vi "UMLEditor loadIniFileInfo.vi"(1 "menu":refnum<k9>, 2 "iniFile":path, 5 "error in (no error)":errorcluster) -> (11 "StabilityProblems":bool, 13 "SyncTime":u32, 15 "Ini-FileFound":bool, 16 "ToolHelp":bool, 17 "LastDiagramType":T1, 18 "FileToOpen":path, 19 "error out":errorcluster)   [LabVIEW 2020]
doc: "Gets current diagram values"
uses:
  <resource>/Framework/Providers/Open_GDS/UML/UMLEditor/UMLEditor_DiagramType.ctl
  <resource>/Framework/Providers/Open_GDS/UML/UMLEditor/UMLEditor_SyncOptions.ctl
  <resource>/Framework/Providers/Open_GDS/UML/UMLEditor/UMLEditor_IniFileData.ctl
  <resource>/Framework/Providers/Open_GDS/UML/UMLEditor/UMLEditor_StoredPathes.ctl
  <resource>/Framework/Providers/Open_GDS/ClassProviders/Common/File/File_StoredPathesActions.ctl
  <resource>/Framework/Providers/Open_GDS/UML/UMLEditor/UMLEditor_StoredColors.ctl
  <resource>/Framework/Providers/Open_GDS/UML/UmlEditor_class/IniParamsType.ctl
  <resource>/Framework/Providers/Open_GDS/ClassProviders/Common/CommonVIs/CommonVIs_ColorMemoryAction.ctl
  <resource>/Framework/Providers/Open_GDS/UML/UMLEditor/UMLEditor MenuActionType.ctl
  <resource>/Framework/Providers/Open_GDS/UML/UmlEditor_class/UmlEditor.lvclass
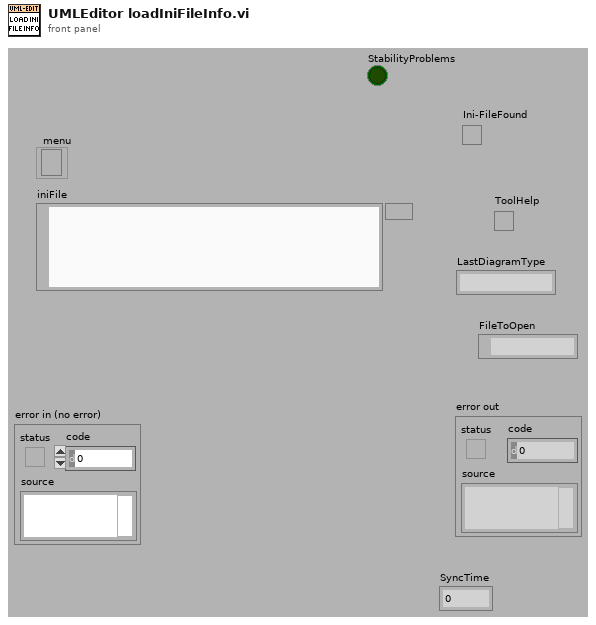
[diagram p1: front panel]
types:
  T1 = typedef "UMLEditor_DiagramType.ctl" = string
  T2 = typedef "UMLEditor_SyncOptions.ctl" = cluster{"IgnoreInstrLib":bool, "IgnoreUserLib":bool, "IgnoreViLib":bool}
  T3 = cluster{"RecentFiles":string[], "LastDiagramType":T1, "ShowToolHelp":bool, "Paths":cluster{"LastSerachPath":path, "QueuedArrayStateVI":path, "ClassBasePath":path, "VITemplatePath":path, "ApplicationTemplatePath":path, "RevPlugIns":path}, "Colors":cluster{"ClassBackgroudColor":u32, "ClassBackgroudColorWithClassPath":u32, "ClassBackgroudColorForApplicationVIStereotype":u32, "ClassBackgroudColorForTypeStereotype":u32, "StateBackgroudColor":u32}, "ProjectBaseClassOption":bool, "CreateTypesWhenSynchronizing":bool, "AttributeToIgnoreInSync":string[], "ToolTip":cluster{"ToolTipOpen":bool, "LastToolTip":i32}, "ClassesToIgnoreInSync":string[], "UndoSize":i32, "OpenLastSavedFile":bool, "SyncOption":T2, "SyncTime":u32, "Params":cluster{"Name":string, "Value":string}[]}
  T4 = typedef "UMLEditor_IniFileData.ctl" = cluster{"RecentFiles":string[], "LastDiagramType":T1, "ShowToolHelp":bool, "Paths":cluster{"LastSerachPath":path, "QueuedArrayStateVI":path, "ClassBasePath":path, "VITemplatePath":path, "ApplicationTemplatePath":path, "RevPlugIns":path}, "Colors":cluster{"ClassBackgroudColor":u32, "ClassBackgroudColorWithClassPath":u32, "ClassBackgroudColorForApplicationVIStereotype":u32, "ClassBackgroudColorForTypeStereotype":u32, "StateBackgroudColor":u32, "ClassBackgroudColorForApplicationInterfaceStereotype":u32}, "ProjectBaseClassOption":bool, "CreateTypesWhenSynchronizing":bool, "AttributeToIgnoreInSync":string[], "ToolTip":cluster{"ToolTipOpen":bool, "LastToolTip":i32}, "ClassesToIgnoreInSync":string[], "UndoSize":i32, "OpenLastSavedFile":bool, "SyncOption":T2, "SyncTime":u32, "Params":cluster{"Name":string, "Value":string}[]}
  T5 = cluster{"RecentFiles":string[], "LastDiagramType":T1, "ShowToolHelp":bool, "Paths":cluster{"LastSerachPath":path, "QueuedArrayStateVI":path, "ClassBasePath":path, "VITemplatePath":path, "ApplicationTemplatePath":path, "RevPlugIns":path}, "Colors":cluster{"ClassBackgroudColor":u32, "ClassBackgroudColorWithClassPath":u32, "ClassBackgroudColorForApplicationVIStereotype":u32, "ClassBackgroudColorForTypeStereotype":u32, "StateBackgroudColor":u32}, "ProjectBaseClassOption":bool, "CreateTypesWhenSynchronizing":bool, "AttributeToIgnoreInSync":string[], "ToolTip":cluster{"ToolTipOpen":bool, "LastToolTip":i32}, "ClassesToIgnoreInSync":string[], "UndoSize":i32, "OpenLastSavedFile":bool, "SyncOption":T2}
  T6 = cluster{"RecentFiles":string[], "LastDiagramType":T1, "ShowToolHelp":bool, "Paths":cluster{"LastSerachPath":path, "QueuedArrayStateVI":path, "ClassBasePath":path, "VITemplatePath":path, "ApplicationTemplatePath":path, "RevPlugIns":path}, "Colors":cluster{"ClassBackgroudColor":u32, "ClassBackgroudColorWithClassPath":u32, "ClassBackgroudColorForApplicationVIStereotype":u32, "ClassBackgroudColorForTypeStereotype":u32, "StateBackgroudColor":u32}, "ProjectBaseClassOption":bool, "CreateTypesWhenSynchronizing":bool, "AttributeToIgnoreInSync":string[], "ToolTip":cluster{"ToolTipOpen":bool, "LastToolTip":i32}, "ClassesToIgnoreInSync":string[], "UndoSize":i32}
  T7 = cluster{"RecentFiles":string[], "LastDiagramType":T1, "ShowToolHelp":bool, "Paths":cluster{"LastSerachPath":path, "QueuedArrayStateVI":path, "ClassBasePath":path, "VITemplatePath":path, "ApplicationTemplatePath":path, "RevPlugIns":path}, "Colors":cluster{"ClassBackgroudColor":u32, "ClassBackgroudColorWithClassPath":u32, "ClassBackgroudColorForApplicationVIStereotype":u32, "ClassBackgroudColorForTypeStereotype":u32, "StateBackgroudColor":u32}, "ProjectBaseClassOption":bool, "CreateTypesWhenSynchronizing":bool, "AttributeToIgnoreInSync":string[], "ToolTip":cluster{"ToolTipOpen":bool, "LastToolTip":i32}, "ClassesToIgnoreInSync":string[], "UndoSize":i32, "OpenLastSavedFile":bool, "SyncOption":T2, "SyncTime":u32}
  T8 = typedef "UmlEditor.lvclass/IniParamsType.ctl" = enum16{"I have problem with UML stability on my computer"}
  T9 = typedef "UMLEditor_StoredColors.ctl" = enum16{"ClassBackgroudColor", "ClassBackgroudColorWithClassPath", "ClassBackgroudColorForApplicationVIStereotype", "ClassBackgroudColorForTypeStereotype", "StateBackgroudColor", "ClassBackgroudColorForInterfaceStereotype"}
  T10 = typedef "UMLEditor_StoredPathes.ctl" = enum16{"LastSearchPath", "QueuedArrayStateVI", "ClassBasePath", "ViTemplatePath", "ApplicationTemplatePath", "IniFilePath", "WizDir", "RevPlugInPath"}
  T11 = typedef "UMLEditor MenuActionType.ctl" = enum16{"EnableSave", "EnablePaste", "DisablePaste", "DiableSave", "AddRecentFile", "disablePropDel", "enablePropDel", "enablePropDisDel", "diasbleClassRel", "enableClassRel", "Class", "State", "Other", "EnableXMI", "DisableXMI", "EnableCopy", "DisableCopy"}
  T12 = typedef "CommonVIs_ColorMemoryAction.ctl" = enum16{"Get Color", "Set Color", "Delete Color", "Clear All Colors"}
  T13 = typedef "File_StoredPathesActions.ctl" = enum16{"Get Path", "Set Path", "Delete Path", "Clear All Paths"}
  T14 = cluster{"LastSerachPath":path, "QueuedArrayStateVI":path, "ClassBasePath":path, "VITemplatePath":path, "ApplicationTemplatePath":path, "RevPlugIns":path}
  T15 = cluster{"ClassBackgroudColor":u32, "ClassBackgroudColorWithClassPath":u32, "ClassBackgroudColorForApplicationVIStereotype":u32, "ClassBackgroudColorForTypeStereotype":u32, "StateBackgroudColor":u32, "ClassBackgroudColorForApplicationInterfaceStereotype":u32}
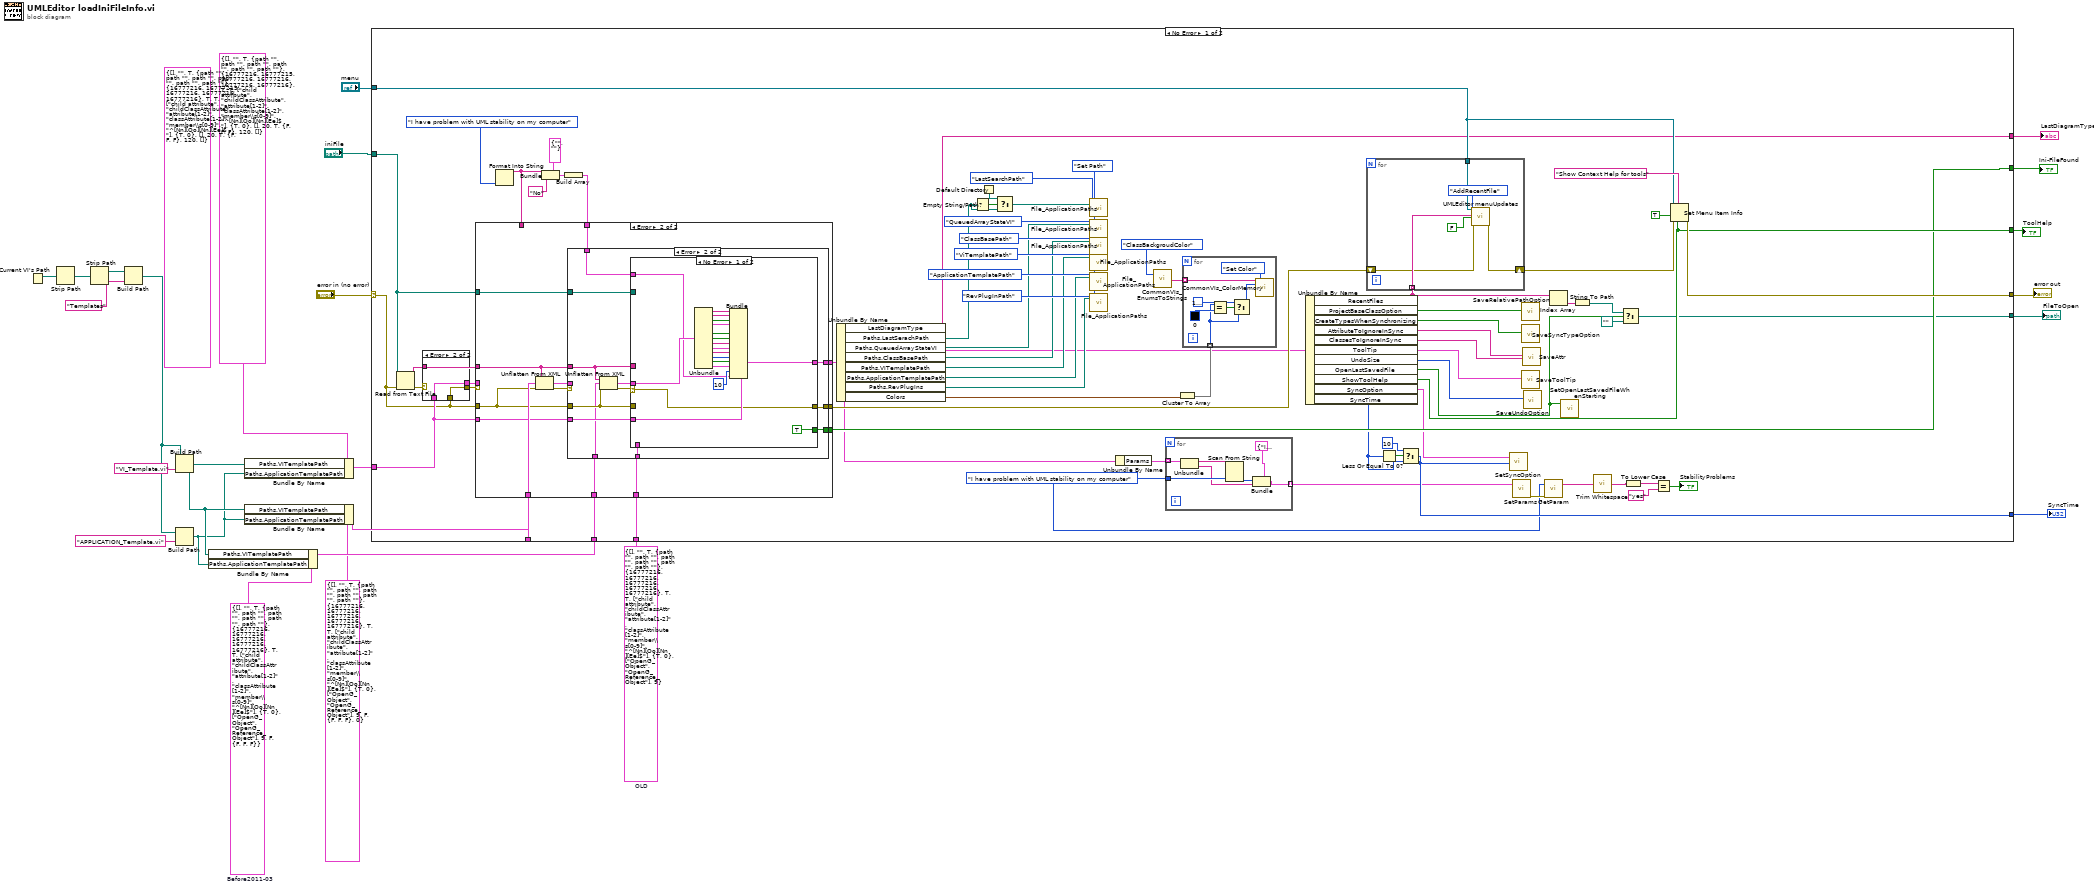
[diagram p0: block diagram]
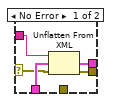
[diagram p2: hidden frame]
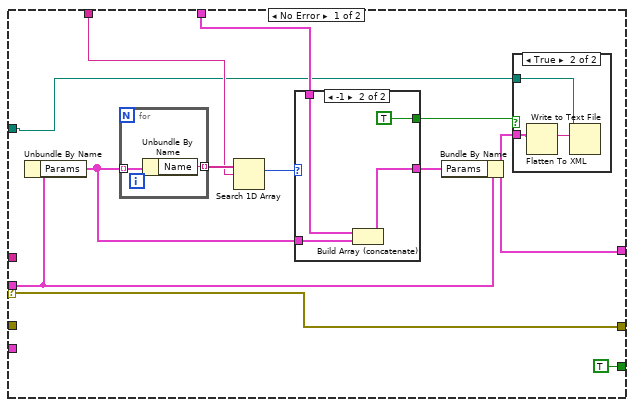
[diagram p3: hidden frame]
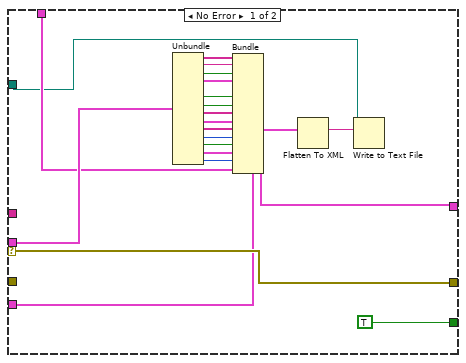
[diagram p6: hidden frame]
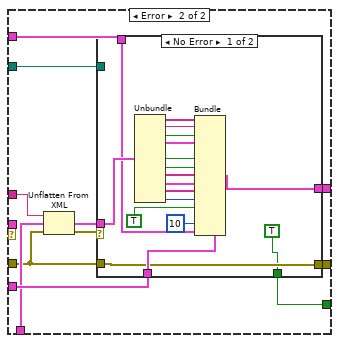
[diagram p7: hidden frame]
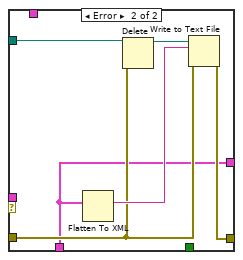
[diagram p8: hidden frame]
diagram:
  (unwired) T3 {"RecentFiles"=[], "LastDiagramType"="", "ShowToolHelp"=TRUE, "Paths"={"LastSerachPath"=path "", "QueuedArrayStateVI"=path "", "ClassBasePath"=path "", "VITemplatePath"=path "", "ApplicationTemplatePath"=path "", "RevPlugIns"=path ""}, "Colors"={"ClassBackgroudColor"=16777216, "ClassBackgroudColorWithClassPath"=16777215, "ClassBackgroudColorForApplicationVIStereotype"=16777216, "ClassBackgroudColorForTypeStereotype"=16777216, "StateBackgroudColor"=16777216}, "ProjectBaseClassOption"=TRUE, "CreateTypesWhenSynchronizing"=TRUE, "AttributeToIgnoreInSync"=["child attribute", "childClassAttribute", "attribute[1-2]", "classAttribute[1-2]", "member\\s[0-9]", "^[Nn][Oo][Nn][Ee]$"], "ToolTip"={"ToolTipOpen"=TRUE, "LastToolTip"=0}, "ClassesToIgnoreInSync"=[], "UndoSize"=20, "OpenLastSavedFile"=TRUE, "SyncOption"={"IgnoreInstrLib"=FALSE, "IgnoreUserLib"=FALSE, "IgnoreViLib"=FALSE}, "SyncTime"=120, "Params"=[]} ("INiFileData")
  w9 = T5 {"RecentFiles"=[], "LastDiagramType"="", "ShowToolHelp"=TRUE, "Paths"={"LastSerachPath"=path "", "QueuedArrayStateVI"=path "", "ClassBasePath"=path "", "VITemplatePath"=path "", "ApplicationTemplatePath"=path "", "RevPlugIns"=path ""}, "Colors"={"ClassBackgroudColor"=16777216, "ClassBackgroudColorWithClassPath"=16777216, "ClassBackgroudColorForApplicationVIStereotype"=16777216, "ClassBackgroudColorForTypeStereotype"=16777216, "StateBackgroudColor"=16777216}, "ProjectBaseClassOption"=TRUE, "CreateTypesWhenSynchronizing"=TRUE, "AttributeToIgnoreInSync"=["child attribute", "childClassAttribute", "attribute[1-2]", "classAttribute[1-2]", "member\\s[0-9]", "^[Nn][Oo][Nn][Ee]$"], "ToolTip"={"ToolTipOpen"=TRUE, "LastToolTip"=0}, "ClassesToIgnoreInSync"=["OpenG_Object", "OpenG_Reference_Object"], "UndoSize"=9, "OpenLastSavedFile"=FALSE, "SyncOption"={"IgnoreInstrLib"=FALSE, "IgnoreUserLib"=FALSE, "IgnoreViLib"=FALSE}}  # Before2011-03
  w11 = T6 {"RecentFiles"=[], "LastDiagramType"="", "ShowToolHelp"=TRUE, "Paths"={"LastSerachPath"=path "", "QueuedArrayStateVI"=path "", "ClassBasePath"=path "", "VITemplatePath"=path "", "ApplicationTemplatePath"=path "", "RevPlugIns"=path ""}, "Colors"={"ClassBackgroudColor"=16777216, "ClassBackgroudColorWithClassPath"=16777216, "ClassBackgroudColorForApplicationVIStereotype"=16777216, "ClassBackgroudColorForTypeStereotype"=16777216, "StateBackgroudColor"=16777216}, "ProjectBaseClassOption"=TRUE, "CreateTypesWhenSynchronizing"=TRUE, "AttributeToIgnoreInSync"=["child attribute", "childClassAttribute", "attribute[1-2]", "classAttribute[1-2]", "member\\s[0-9]", "^[Nn][Oo][Nn][Ee]$"], "ToolTip"={"ToolTipOpen"=TRUE, "LastToolTip"=0}, "ClassesToIgnoreInSync"=["OpenG_Object", "OpenG_Reference_Object"], "UndoSize"=9}  # OLD
  n1 = Current VI's Path() -> (path=w18:path)
  n2 = Strip Path(path=w18) -> (stripped path=w17:path)  [unwired: 1 out]
  n3 = Strip Path(path=w17) -> (stripped path=w16:path)  [unwired: 1 out]
  n4 = Build Path(base path=w16, name or relative path="Templates") -> (appended path=w14:path)
  n5 = Build Path(base path=w14, name or relative path="VI_Template.vi") -> (appended path=w5:path)
  n6 = Build Path(base path=w14, name or relative path="APPLICATION_Template.vi") -> (appended path=w4:path)
  n7 = Bundle By Name(cluster=w9, "Paths.VITemplatePath"=w5, "Paths.ApplicationTemplatePath"=w4) -> (w8:T5)
  n8 = Bundle By Name(cluster=T4 {"RecentFiles"=[], "LastDiagramType"="", "ShowToolHelp"=TRUE, "Paths"={"LastSerachPath"=path "", "QueuedArrayStateVI"=path "", "ClassBasePath"=path "", "VITemplatePath"=path "", "ApplicationTemplatePath"=path "", "RevPlugIns"=path ""}, "Colors"={"ClassBackgroudColor"=16777216, "ClassBackgroudColorWithClassPath"=16777215, "ClassBackgroudColorForApplicationVIStereotype"=16777216, "ClassBackgroudColorForTypeStereotype"=16777216, "StateBackgroudColor"=16777216, "ClassBackgroudColorForApplicationInterfaceStereotype"=16777216}, "ProjectBaseClassOption"=TRUE, "CreateTypesWhenSynchronizing"=TRUE, "AttributeToIgnoreInSync"=["child attribute", "childClassAttribute", "attribute[1-2]", "classAttribute[1-2]", "member\\s[0-9]", "^[Nn][Oo][Nn][Ee]$"], "ToolTip"={"ToolTipOpen"=TRUE, "LastToolTip"=0}, "ClassesToIgnoreInSync"=[], "UndoSize"=20, "OpenLastSavedFile"=TRUE, "SyncOption"={"IgnoreInstrLib"=FALSE, "IgnoreUserLib"=FALSE, "IgnoreViLib"=FALSE}, "SyncTime"=120, "Params"=[]} ("INiFileData"), "Paths.VITemplatePath"=w5, "Paths.ApplicationTemplatePath"=w4) -> (w3:T4)
  n9 = Bundle By Name(cluster=T7 {"RecentFiles"=[], "LastDiagramType"="", "ShowToolHelp"=TRUE, "Paths"={"LastSerachPath"=path "", "QueuedArrayStateVI"=path "", "ClassBasePath"=path "", "VITemplatePath"=path "", "ApplicationTemplatePath"=path "", "RevPlugIns"=path ""}, "Colors"={"ClassBackgroudColor"=16777216, "ClassBackgroudColorWithClassPath"=16777216, "ClassBackgroudColorForApplicationVIStereotype"=16777216, "ClassBackgroudColorForTypeStereotype"=16777216, "StateBackgroudColor"=16777216}, "ProjectBaseClassOption"=TRUE, "CreateTypesWhenSynchronizing"=TRUE, "AttributeToIgnoreInSync"=["child attribute", "childClassAttribute", "attribute[1-2]", "classAttribute[1-2]", "member\\s[0-9]", "^[Nn][Oo][Nn][Ee]$"], "ToolTip"={"ToolTipOpen"=TRUE, "LastToolTip"=0}, "ClassesToIgnoreInSync"=["OpenG_Object", "OpenG_Reference_Object"], "UndoSize"=9, "OpenLastSavedFile"=FALSE, "SyncOption"={"IgnoreInstrLib"=FALSE, "IgnoreUserLib"=FALSE, "IgnoreViLib"=FALSE}, "SyncTime"=0} ("INiFileData"), "Paths.VITemplatePath"=w5, "Paths.ApplicationTemplatePath"=w4) -> (w19:T7)
  n10 = case shown="No Error" "error in (no error)" {
    selector: "error in (no error)" -> [w27 w247]
    tunnel: [w97 w247] -> w24
    tunnel: [w65 _] -> w23
    tunnel: [w71 _] -> w22
    tunnel: [w26 _] -> w21
    tunnel: "menu" -> [w94 _]
    tunnel: "iniFile" -> [w80 _]
    tunnel: w19 -> [w81 _]
    tunnel: w11 -> [w61 _]
    tunnel: [w55 _] -> w10
    tunnel: w8 -> [w53 _]
    tunnel: [w50 _] -> w7
    tunnel: w3 -> [w45 _]
    frame No Error {
      w35 = IniParamsType."I have problem with UML stability on my computer" ("IniParams")
      w84 = File_StoredPathesActions."Set Path" ("Method (Get Path)")
      n11 = Read from Text File(file (use dialog)=w80, error in=w27) -> (text=w48:string, error out=w28:errorcluster)  [unwired: 4 out]
      n12 = case shown="Error" w28 {
        selector: w28 -> [w98 _]
        tunnel: w48 -> [w102 _]
        tunnel: [w101 w103] -> w47
        tunnel: [w100 w104] -> w46
        tunnel: w45 -> [w99 w104]
        tunnel: w27 -> [_ w103]
        frame No Error {
          n13 = Unflatten From XML(xml string=w102, type=w99, error in (no error)=w98) -> (value=w100:T4, error out=w101:errorcluster)
        }
        frame Error {
        }
      }
      n14 = Format Into String(IniParamsType."I have problem with UML stability on my computer" ("IniParams")) -> (resulting string=w29:string)  [unwired: 3 in, 1 out]
      n15 = Bundle(cluster=cluster{"Name":string, "Value":string} {"Name"="", "Value"=""} ("Param"), "Name"=w29, "Value"="No") -> (w41:cluster{"Name":string, "Value":string})
      n16 = Build Array(w41) -> (w40:cluster{"Name":string, "Value":string}[])
      n17 = case shown="Error" w47 {
        selector: w47 -> [w123 _]
        tunnel: w27 -> [_ w136]
        tunnel: w81 -> [_ w145]
        tunnel: w80 -> [w113 w144]
        tunnel: [w123 w142] -> w70
        tunnel: [TRUE w141] -> w65
        tunnel: w61 -> [_ w140]
        tunnel: [w112 w139] -> w39
        tunnel: w53 -> [_ w138]
        tunnel: w48 -> [_ w137]
        tunnel: w46 -> [w119 _]
        tunnel: w45 -> [_ w135]
        tunnel: w40 -> [w116 w134]
        tunnel: w29 -> [w120 _]
        frame No Error {
          n18 = Unbundle By Name(w119) -> ("Params"=w117:cluster{"Name":string, "Value":string}[])
          n19 = for {
            tunnel: w117 -> [w133] mode=indexing
            tunnel: [w132] -> w121 mode=indexing
            n20 = Unbundle By Name(w133) -> ("Name"=w132:string)
          }
          n21 = Search 1D Array(1D array=w121, element=w120) -> (index of element=w118:i32)  [unwired: 1 in]
          n22 = case shown="-1" w118 {
            tunnel: w117 -> [w127 w131]
            tunnel: w116 -> [_ w130]
            tunnel: [w127 w129] -> w115
            tunnel: [_ TRUE] -> w114
            frame 0, Default {
            }
            frame -1 {
              n23 = Build Array (concatenate)(w130, w131) -> (w129:cluster{"Name":string, "Value":string}[])
            }
          }
          n24 = Bundle By Name(cluster=w119, "Params"=w115) -> (w112:T4)
          n25 = case shown="True" w114 {
            tunnel: w113 -> [_ w125]
            tunnel: w112 -> [_ w124]
            frame False {
            }
            frame True {
              n26 = Flatten To XML(6:w124) -> (2:w126:string)
              n27 = Write to Text File(file (use dialog)=w125, text=w126) -> ()  [unwired: 1 in, 4 out]
            }
          }
        }
        frame Error {
          n28 = Unflatten From XML(xml string=w137, type=w145, error in (no error)=w136) -> (value=w143:T7, error out=w146:errorcluster)
          n29 = case shown="Error" w146 {
            selector: w146 -> [w167 _]
            tunnel: [w167 w177] -> w142
            tunnel: w136 -> [_ w173]
            tunnel: w135 -> [w151 w178]
            tunnel: w144 -> [w147 w179]
            tunnel: w143 -> [w153 _]
            tunnel: [TRUE w176] -> w141
            tunnel: w137 -> [_ w172]
            tunnel: w140 -> [_ w175]
            tunnel: [w149 w174] -> w139
            tunnel: w138 -> [_ w169]
            tunnel: w134 -> [w150 w168]
            frame No Error {
              n30 = Unbundle(w153) -> ("RecentFiles"=w165:string[], "LastDiagramType"=w164:T1, "ShowToolHelp"=w163:bool, "Paths"=w162:T14, "ProjectBaseClassOption"=w161:bool, "CreateTypesWhenSynchronizing"=w160:bool, "AttributeToIgnoreInSync"=w159:string[], "ToolTip"=w158:cluster{"ToolTipOpen":bool, "LastToolTip":i32}, "ClassesToIgnoreInSync"=w157:string[], "UndoSize"=w156:i32, "OpenLastSavedFile"=w155:bool, "SyncOption"=w154:T2, "SyncTime"=w152:u32)  [unwired: 1 out]
              n31 = Bundle(cluster=w151, "RecentFiles"=w165, "LastDiagramType"=w164, "ShowToolHelp"=w163, "Paths"=w162, "ProjectBaseClassOption"=w161, "CreateTypesWhenSynchronizing"=w160, "AttributeToIgnoreInSync"=w159, "ToolTip"=w158, "ClassesToIgnoreInSync"=w157, "UndoSize"=w156, "OpenLastSavedFile"=w155, "SyncOption"=w154, "SyncTime"=w152, "Params"=w150) -> (w149:T4)  [unwired: 1 in]
              n32 = Flatten To XML(6:w149) -> (2:w148:string)
              n33 = Write to Text File(file (use dialog)=w147, text=w148) -> ()  [unwired: 1 in, 4 out]
            }
            frame Error {
              n34 = Unflatten From XML(xml string=w172, type=w169, error in (no error)=w173) -> (value=w170:T5, error out=w171:errorcluster)
              n35 = case shown="No Error" w171 {
                selector: w171 -> [w182 _]
                tunnel: w179 -> [_ w209]
                tunnel: w178 -> [w185 w208]
                tunnel: [w182 w207] -> w177
                tunnel: [TRUE w200] -> w176
                tunnel: w175 -> [_ w206]
                tunnel: [w183 w203] -> w174
                tunnel: w173 -> [_ w202]
                tunnel: w172 -> [_ w201]
                tunnel: w170 -> [w188 _]
                tunnel: w168 -> [w180 w199]
                frame No Error {
                  n36 = Unbundle(w188) -> ("RecentFiles"=w198:string[], "LastDiagramType"=w197:T1, "ShowToolHelp"=w196:bool, "Paths"=w195:T14, "ProjectBaseClassOption"=w194:bool, "CreateTypesWhenSynchronizing"=w193:bool, "AttributeToIgnoreInSync"=w192:string[], "ToolTip"=w191:cluster{"ToolTipOpen":bool, "LastToolTip":i32}, "ClassesToIgnoreInSync"=w190:string[], "UndoSize"=w189:i32, "OpenLastSavedFile"=w187:bool, "SyncOption"=w186:T2)  [unwired: 1 out]
                  n37 = Bundle(cluster=w185, "RecentFiles"=w198, "LastDiagramType"=w197, "ShowToolHelp"=w196, "Paths"=w195, "ProjectBaseClassOption"=w194, "CreateTypesWhenSynchronizing"=w193, "AttributeToIgnoreInSync"=w192, "ToolTip"=w191, "ClassesToIgnoreInSync"=w190, "UndoSize"=w189, "OpenLastSavedFile"=w187, "SyncOption"=w186, "SyncTime"=u32 10, "Params"=w180) -> (w183:T4)  [unwired: 1 in]
                }
                frame Error {
                  n38 = Unflatten From XML(xml string=w201, type=w206, error in (no error)=w202) -> (value=w204:T6, error out=w205:errorcluster)
                  n39 = case shown="No Error" w205 {
                    tunnel: w209 -> [_ w233]
                    tunnel: w208 -> [w226 w228]
                    tunnel: [w213 w229] -> w207
                    tunnel: w202 -> [w213 w230]
                    tunnel: w204 -> [w227 _]
                    tunnel: [w214 w228] -> w203
                    tunnel: [TRUE _] -> w200
                    tunnel: w199 -> [w210 _]
                    frame No Error {
                      n40 = Unbundle(w227) -> ("RecentFiles"=w225:string[], "LastDiagramType"=w224:T1, "ShowToolHelp"=w223:bool, "Paths"=w222:T14, "ProjectBaseClassOption"=w221:bool, "CreateTypesWhenSynchronizing"=w220:bool, "AttributeToIgnoreInSync"=w219:string[], "ToolTip"=w218:cluster{"ToolTipOpen":bool, "LastToolTip":i32}, "ClassesToIgnoreInSync"=w217:string[], "UndoSize"=w216:i32)  [unwired: 1 out]
                      n41 = Bundle(cluster=w226, "RecentFiles"=w225, "LastDiagramType"=w224, "ShowToolHelp"=w223, "Paths"=w222, "ProjectBaseClassOption"=w221, "CreateTypesWhenSynchronizing"=w220, "AttributeToIgnoreInSync"=w219, "ToolTip"=w218, "ClassesToIgnoreInSync"=w217, "UndoSize"=w216, "OpenLastSavedFile"=TRUE, "SyncTime"=u32 10, "Params"=w210) -> (w214:T4)  [unwired: 2 in]
                    }
                    frame Error {
                      n42 = Flatten To XML(6:w228) -> (2:w231:string)
                      n43 = Delete(path (use dialog)=w233, error in=w230) -> (deleted path=w232:path)  [unwired: 5 out]
                      n44 = Write to Text File(file (use dialog)=w232, text=w231, error in=w230) -> (error out=w229:errorcluster)  [unwired: 3 out]
                    }
                  }
                }
              }
            }
          }
        }
      }
      n45 = Unbundle By Name(w39) -> ("LastDiagramType"=w26:T1, "Paths.LastSerachPath"=w79:path, "Paths.QueuedArrayStateVI"=w78:path, "Paths.ClassBasePath"=w77:path, "Paths.VITemplatePath"=w76:path, "Paths.ApplicationTemplatePath"=w74:path, "Paths.RevPlugIns"=w75:path, "Colors"=w73:T15)
      n46 = Empty String/Path?(string/path=w79) -> (empty?=w92:bool)
      n47 = Default Directory() -> (w91:path)
      n48 = Select(t=w91, s=w92, f=w79) -> (s? t:f=w88:path)
      n49 = call <resource>:"File_ApplicationPaths.vi"("PathName"=UMLEditor_StoredPathes."LastSearchPath" ("UMLPathes"), "Path In"=w88, "Method (Get Path)"=w84) -> ()  [unwired: 1 in, 16 out]
      n50 = call <resource>:"File_ApplicationPaths.vi"("PathName"=UMLEditor_StoredPathes."QueuedArrayStateVI" ("UMLPathes"), "Path In"=w78, "Method (Get Path)"=w84) -> ()  [unwired: 1 in, 16 out]
      n51 = call <resource>:"File_ApplicationPaths.vi"("PathName"=UMLEditor_StoredPathes."ClassBasePath" ("UMLPathes"), "Path In"=w77, "Method (Get Path)"=w84) -> ()  [unwired: 1 in, 16 out]
      n52 = call <resource>:"File_ApplicationPaths.vi"("PathName"=UMLEditor_StoredPathes."ViTemplatePath" ("UMLPathes"), "Path In"=w76, "Method (Get Path)"=w84) -> ()  [unwired: 1 in, 16 out]
      n53 = call <resource>:"File_ApplicationPaths.vi"("PathName"=UMLEditor_StoredPathes."ApplicationTemplatePath" ("UMLPathes"), "Path In"=w74, "Method (Get Path)"=w84) -> ()  [unwired: 1 in, 16 out]
      n54 = call <resource>:"File_ApplicationPaths.vi"("PathName"=UMLEditor_StoredPathes."RevPlugInPath" ("UMLPathes"), "Path In"=w75, "Method (Get Path)"=w84) -> ()  [unwired: 1 in, 16 out]
      n55 = Unbundle By Name(w39) -> ("Params"=w38:cluster{"Name":string, "Value":string}[])
      n56 = call <resource>:"CommonVIs_EnumsToStrings.vi"("ArrayEnumVariantIn"=UMLEditor_StoredColors."ClassBackgroudColor" ("UMLPathes")) -> ("EnumChoices"=w82:string[])  [unwired: 2 in, 16 out]
      n57 = for {
        tunnel: w38 -> [w110] mode=indexing
        tunnel: w35 -> [w109]
        tunnel: [w105] -> w37 mode=indexing
        n58 = Unbundle(w110) -> ("Name"=w108:string, "Value"=w106:string)
        n59 = Scan From String(input string=w108, default 1=w109) -> (output 1=w107:T8)  [unwired: 3 in, 3 out]
        n60 = Bundle(cluster=cluster{"IniParams":T8, "Value":string} {"IniParams"=enum."I have problem with UML stability on my computer", "Value"=""} ("Param"), "IniParams"=w107, "Value"=w106) -> (w105:cluster{"IniParams":T8, "Value":string})
      }
      n61 = Cluster To Array(cluster=w73) -> (array=w72:u32[])
      n62 = for {
        tunnel: w82 -> [w245] mode=indexing
        tunnel: w72 -> [w240] mode=indexing
        n63 = Equal?(x=w240, y=u32 0) -> (x = y?=w243:bool)
        n64 = Select(t=u32 16777216, s=w243, f=w240) -> (s? t:f=w241:u32)
        n65 = call <resource>:"CommonVIs_ColorMemory.vi"("ColorName"=w245, "Color In"=w241, "Method (Get Color)"=CommonVIs_ColorMemoryAction."Set Color") -> ()  [unwired: 1 in, 16 out]
      }
      n66 = Unbundle By Name(w39) -> ("RecentFiles"=w59:string[], "ProjectBaseClassOption"=w69:bool, "CreateTypesWhenSynchronizing"=w68:bool, "AttributeToIgnoreInSync"=w67:string[], "ClassesToIgnoreInSync"=w63:string[], "ToolTip"=w64:cluster{"ToolTipOpen":bool, "LastToolTip":i32}, "UndoSize"=w62:i32, "OpenLastSavedFile"=w60:bool, "ShowToolHelp"=w71:bool, "SyncOption"=w54:T2, "SyncTime"=w51:u32)
      n67 = for {
        shift-right: [w239] -> w66
        shift-left: w70 -> [w234]
        tunnel: w94 -> [w238]
        tunnel: w59 -> [w237] mode=indexing
        n68 = call <resource>:"UMLEditor menuUpdates.vi"("menu"=w238, "menuAction"=UMLEditor_MenuActionType."AddRecentFile", "item"=w237, "addfirst(false)"=FALSE, "error in (no error)"=w234) -> ("error out"=w239:errorcluster)  [unwired: 1 in, 13 out]
      }
      n69 = Less Or Equal To 0?(x=w51) -> (x <= 0?=w52:bool)
      n70 = Select(t=u32 10, s=w52, f=w51) -> (s? t:f=w50:u32)
      n71 = call <resource>:"SetSyncOption.vi"("SyncOption"=w54, "SyncTime(s)"=w50) -> ()  [unwired: 17 in, 1 out]
      n72 = call <resource>:"SetParams.vi"("Params"=w37) -> ("error out"=w36:errorcluster)  [unwired: 18 in]
      n73 = call <resource>:"SaveRelativePathOption.vi"("UseProjectFolderAsBasePath"=w69) -> ()  [unwired: 1 in, 18 out]
      n74 = call <resource>:"SaveSyncTypeOption.vi"("TypeSyncOption"=w68) -> ()  [unwired: 1 in, 18 out]
      n75 = call <resource>:"SaveToolTip.vi"("ToolTip"=w64) -> ()  [unwired: 1 in, 18 out]
      n76 = call <resource>:"SaveAttr.vi"("AttrToIgnore"=w67, "ClassesToIgnore"=w63) -> ()  [unwired: 1 in, 17 out]
      n77 = call <resource>:"SaveUndoOption.vi"("UndoSize"=w62) -> ()  [unwired: 1 in, 18 out]
      n78 = call <resource>:"GetParam.vi"("IniParams"=w35, "error in (no error)"=w36) -> ("Value"=w34:string)  [unwired: 15 in, 2 out]
      n79 = Index Array(array=w59) -> (element=w58:string)  [unwired: 1 in]
      n80 = call <resource>:"SetOpenLastSavedFileWhenStarting.vi"("OpenLastSavedFileWhenStarting"=w60) -> ()  [unwired: 18 in, 1 out]
      n81 = String To Path(string=w58) -> (path=w57:path)
      n82 = call <vilib>:"Trim Whitespace.vi"("string"=w34) -> ("trimmed string"=w33:string)  [unwired: 1 in]
      n83 = Select(t=w57, s=w60, f=path "") -> (s? t:f=w55:path)
      n84 = To Lower Case(string=w33) -> (all lower case string=w32:string)
      n85 = Equal?(x=w32, y="yes") -> (x = y?=→"StabilityProblems":bool)
      n86 = Set Menu Item Info(6:w71, 7:"Show Context Help for tools" ("item tag"), 8:w66, 9:TRUE ("enabled"), 11:w94) -> (0:w97:errorcluster)  [unwired: 3 out]
    }
    frame Error {
    }
  }
  "error out" <- w24
  "Ini-FileFound" <- w23
  "ToolHelp" <- w22
  "LastDiagramType" <- w21
  "FileToOpen" <- w10
  "SyncTime" <- w7
